vi "AlliGator Decay Fit Parameter Map Panel.vi"() -> ()   [LabVIEW 2021, in "AlliGator Decay Fit Parameter Map.lvlib"]
uses:
  AlliGator Decay Fit Parameter Map.lvlib
  Fits/IRF(X)PSED/Decay Fit Parameters & Derived Quantities List v2.ctl
  AlliGator Decay Fit Parameter Map Control Refnums.ctl
  Globals, Variables, Constants/AlliGator Refnums List.ctl
  Utilities/Read-Write.ctl
  Settings/AlliGator Settings List.ctl
  Action Engine/AlliGator Q Element.ctl
  Action Engine/AlliGator Q Event.ctl
  Globals, Variables, Constants/AlliGator Variables List.ctl
  Palette/Image Palette Information.ctl
  Image/Image Display Palette Type.ctl
  Image/Image Display Event.ctl
  Image/Image Control Refnum.ctl
  <vilib>/Utility/miscctls.llb/LVPoint32TypeDef.ctl
  AlliGator Decay Parameter Map Update Event Data.ctl
  GUI/AlliGator Image Mouse Up Event Data.ctl
  Image/Image ROI Descriptor.ctl
  Image/Image Contour Definition.ctl
  Image/Image Contour ID.ctl
  Image/Image ROI Type.ctl
  Variant/Variant to Data/Variant to Boolean.vi
  Variant/Variant to Data/Variant to [String].vi
  Settings/AlliGator Settings+.lvlib
  Variant/Variant to Data/Variant to Data.lvlib
  Notebook/Notebook.lvlib
  Action Engine/AlliGator Action Engine.lvlib
  GUI/GUI.lvlib
  GUI/AlliGator GUI.lvlib
  Error/Error.lvlib
  Image/Image.lvlib
  Palette/Palette.lvlib
  Globals, Variables, Constants/AlliGator Globals, Variables & Constants.lvlib
  Python Plugins API/AlliGator Python Plugins.lvlib
  Phasor Plot/AlliGator Phasor Plot.lvlib
  Fits/Fits.lvlib
  Utilities/Utilities.lvlib
panel:
  in  "Decay Fit Parameter":T1
  in  "Pin Button":bool=TRUE
  in  "Overlay Decay Fit Parameter Map":bool
  in  "Decay Fit Parameter ROI Color":u32(colorbox)=6618880 caption="Phasor Plot ROI Color"
  in  "Refresh Decay Fit Parameter Map":bool caption="Refresh Phsor Plot"
  out "Decay Fit Parameter Map Display":T2(plugin-control)
  out "Decay Parameter Map Value":dbl caption="Map Value" format="%#_5e"
  out "Decay Parameter Map Y":i32 caption="Y"
  out "Decay Parameter Map X":i32 caption="X"
  out "Decay Fit Min Parameter":dbl caption="Min Parameter" format="%#_5e"
  out "Decay Fit Max Parameter":dbl=1.0 caption="Max Parameter" format="%#_5e"
  in  "Decay Fit Parameter Map Color Scale":dbl(ramp)
  in  "Decay Fit Parameter Map Display Range":cluster{dbl, dbl}(slide)={0.0, 1.0} scale=0.7838060855865479..1.044173002243042 scale format="%04_3g"
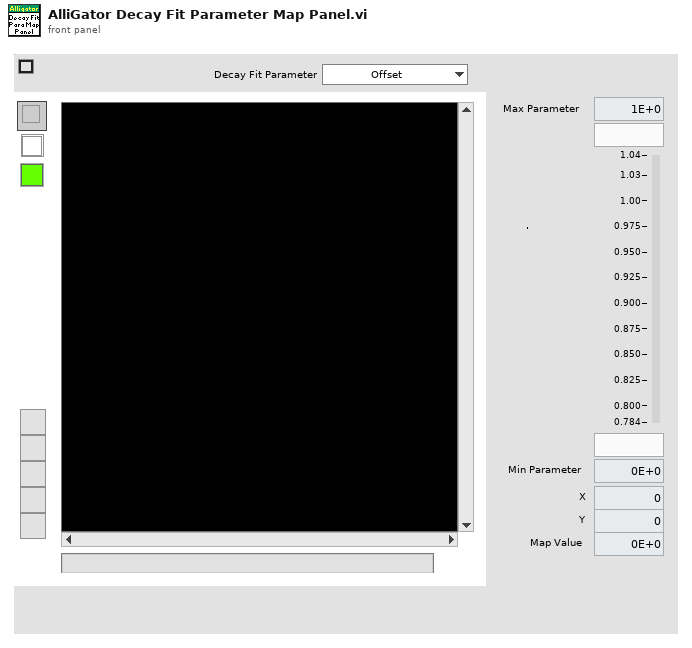
[diagram p1: front panel]
types:
  T1 = typedef "Fits.lvlib/Decay Fit Parameters & Derived Quantities List v2.ctl" = enum16{"Offset", "Baseline", "A_1", "tau_1", "A_2", "tau_2", "<tau>_a", "f1_a", "f2_a", "<tau>_i", "f1_i", "f2_i", "-", "R^2", "Chi^2"}
  T2 = typedef "IMAQ Image.ctl" = refnum<image>
  T3 = typedef "Utilities.lvlib/Read-Write.ctl" = enum16{"Read", "Write"}
  T4 = typedef "AlliGator GUI.lvlib/AlliGator Refnums List.ctl" = enum16{"---------- AlliGator Control Refnums ----------", "AlliGator Tab Control Refnum", "Dataset Ctrl Refnums", "Image Histogram Ctrl Refnums", "Intensity Time Trace Ctrl Refnums", "Decay Graph Ctrl Refnums", "Decay Statistics Graph Ctrl Refnums", "Phasor Graph Ctrl Refnums", "Phasor Ratio Graph Ctrl Refnums", "Phasor Plot Ctrl Refnums", "Lifetime & Other Parameters Ctrl Refnums", "Decay Fit Parameter Map Ctrl Refnums", "Parameter Map Ctrl Refnums", "Other AlliGator Ctrl Refnums", "---------- AlliGator Menu Refnums ----------", "AlliGator Menu", "---------- IO Device ID ----------", "Mouse ID", "Keyboard ID"}
  T5 = typedef "AlliGator Decay Fit Parameter Map.lvlib/AlliGator Decay Fit Parameter Map Control Refnums.ctl" = cluster{"Decay Fit Parameter Map Color Scale":refnum<vi>, "Decay Fit Parameter":refnum<vi>, "Max Parameter":refnum<vi>, "Min Parameter":refnum<vi>, "Decay Fit Parameter Map Display":refnum<vi>, "Decay Fit Parameter Map Display Range":refnum<vi>, "Decay Parameter Map X":refnum<vi>, "Decay Parameter Map Y":refnum<vi>, "Decay Parameter Map Value":refnum<vi>}
  T6 = cluster{"Event Registration Refnum":refnum<event-registration>, "Decay Fit Parameter Map Display Range Event":refnum<event-registration>, "Decay Fit Parameter Map Display Event":refnum<event-registration>}
  T7 = typedef "AlliGator Settings+.lvlib/AlliGator Settings List.ctl" = enum16{"GUI:Visible Settings Tab", "GUI:Last Run Version", "Source Image:Use Image Histogram for Contrast", "Source Image:Low Count Pixels Rejection Options", "Source Image:High Count Pixels Rejection Options", "Source Image:Use Image Brightness", "Source Image:Blend Overlay with Image Background", "Source Image:Use Fixed ROI Diameter", "Source Image:ROI Diameter", "Source Image:ROI Center Color", "Source Image:Peak Threshold", "Source Image:Intensity Threshold", "Source Image:Image Binning Options", "Source Image:Image Smoothing Options", "Source Image:Image Histogram Active", "Source Image:Invert Binary Mask", "Source Image:Hot Pixel Removal", "Source Image:Overlay Analyzed ROI Center", "Source Image:Auto-Adjust Contrast", "Source Image:Histogram Lower Percentile", "Source Image:Histogram Upper Percentile", "Source Image:Lock ROI with Maps", "Source Image:Save Source Image", "Source Image:Scale Bar Options", "Source Image:Image Resolution (Pixel Size)", "Source Image:Flatfield Correction", "Source Image:Show Dead Left Columns Correction", "Source Image:Dead Left Columns Correction", "Source Image:Image Pre-Processing Operations Order", "Source Image:Overlay ROI Median", "Source Image:Median Overlay Color", "Data Information:Gate Width", "Data Information:Nanotime Gate Separation", "Data Information:Macrotime Gate Separation", "Data Information:Gate Step", "Data Information:# Gates", "Data Information:Gate Image Exposure", "Data Information:Gate Image Integration", "Data Information:Gates to Skip", "Data Information:Gates to Keep", "Data Information:Define Gates to", "Data Information:Channel Name", "Data Information:Available Channel Names", "Data Information:Channel Arithmetic", "Data Information:Background File Subtraction", "Data Information:Background File", "Data Information:Background Scaling Factor", "Data Information:Background Pile-up Correction", "Data Information:Background Pixel Well Capacity", "Data Information:Laser Period", "Data Information:SYNC Period", "Data Information:Pile-up Correction", "Data Information:Pixel Well Capacity", "Data Information:Dataset Scaling Factor", "Fluorescence Decay_Decay Pre-Processing:Reverse Gates", "Fluorescence Decay_Decay Pre-Processing:Verbose Decay Pre-Processing", "Fluorescence Decay_Decay Pre-Processing:Use Decay Pre-Processing", "Fluorescence Decay_Decay Pre-Processing:Background Subtraction", "Fluorescence Decay_Decay Pre-Processing:Background Definition Range", "Fluorescence Decay_Decay Pre-Processing:Baseline Subtraction Method", "Fluorescence Decay_Decay Pre-Processing:Decay Pre-Processing Operations Order", "Fluorescence Decay_Decay Pre-Processing:Smoothing Parameter", "Fluorescence Decay_Decay Pre-Processing:Shift Decay", "Fluorescence Decay_Decay Pre-Processing:Decay Shift Parameters", "Fluorescence Decay_Decay Pre-Processing:Fold Decay", "Fluorescence Decay_Decay Pre-Processing:# Folds", "Fluorescence Decay_Decay Pre-Processing:1-Normalize Decay", "Fluorescence Decay_Decay Pre-Processing:[0-1]-Normalize Decay", "Fluorescence Decay_Decay Pre-Processing:Smoothen Decay", "Fluorescence Decay_Decay Pre-Processing:Extrapolate Decay", "Fluorescence Decay_Decay Pre-Processing:Use Periodicity", "Fluorescence Decay_Decay Pre-Processing:Use Cursors", "Fluorescence Decay_Decay Pre-Processing:Tail Fraction", "Fluorescence Decay_Decay Pre-Processing:Head Fraction", "Fluorescence Decay_Decay Pre-Processing:Additional Points", "Fluorescence Decay_Decay Pre-Processing:Straighten Decay", "Fluorescence Decay_Decay Pre-Processing:Constant Background", "Fluorescence Decay_Decay Pre-Processing:Pixel-Normalize Decay", "Fluorescence Decay_Advanced Analysis:Extract IRF instead of Decay", "Fluorescence Decay_Advanced Analysis:IRF Extraction Options", "Fluorescence Decay_Advanced Analysis:IRF Optimization Options", "Fluorescence Decay_Advanced Analysis:Square Pulse Options", "Fluorescence Decay_Advanced Analysis:IRF Order", "Fluorescence Decay_Advanced Analysis:IRF Time Constants", "Fluorescence Decay_Advanced Analysis:Wavelet Analysis Options", "Fluorescence Decay_Advanced Analysis:Average Lifetime Options", "Fluorescence Decay_Fit Options:Fit Options", "Fluorescence Decay_Fit Options:Use Legacy Fitting Approach", "Fluorescence Decay_Fit Options:Use Data Information Laser Period", "Fluorescence Decay_Fit Parameters:Displayed Fit Parameters", "Fluorescence Decay_Fit Parameters:Fit Parameter Constraints", "Fluorescence Decay_Fit Parameters:Export Tabulated Results", "Fluorescence Decay_Fit Parameters:MLE Baseline Offset Type", "Fluorescence Decay_Fit Parameters:MLE Baseline Offset", "Fluorescence Decay_Fit Parameters:Guess Parameter Names", "Fluorescence Decay_Fit Parameters:Guess Parameter Values", "Fluorescence Decay_Fit Parameters:Guess Parameters Options", "Fluorescence Decay_Fit Parameters:Optimal Offset Selection Criterion", "Fluorescence Decay_Styles:Show Last Decay Only", "Fluorescence Decay_Styles:Decay Graph Color Array", "Fluorescence Decay:Decay Graph Active", "Fluorescence Decay Statistics:Min Peak Value", "Fluorescence Decay Statistics:Reject Low Decay Peak Pixels", "Fluorescence Decay Statistics:Reject High Decay Peak Pixels", "Fluorescence Decay Statistics:Max Peak Value", "Time Traces:Use File Timestamp", "Time Traces:Time Step", "Time Traces:Use Intensity Correction File", "Time Traces:Intensity Correction File", "Phasor Plot:Phasor Plot Smoothing Options", "Phasor Plot:Phasor Plot Size", "Phasor Plot:Phasor Plot Graphics Options", "Phasor Plot:Cumulative Phasor Plot", "Phasor Plot:Use Phasor Brightness", "Phasor Plot:Blend Overlay with Phasor Background", "Phasor Plot:Save Phasor Plot", "Phasor Plot:Show References", "Phasor Plot:Phasor Ratio Decay Range", "Phasor Plot:Exponential Fading", "Phasor Plot:Phasor Ratio Reference Colors", "Phasor Plot:Reference Radius", "Phasor Plot:Show Color Map Vertices", "Phasor Plot:Phasor Plot Active", "Phasor Plot:Phasor Ratio Color Map Type", "Phasor Plot:Phasor Ratio Color Map", "Phasor Plot:Phasor Ratio Display Range", "Phasor Plot:Selected Image ROI(s)", "Phasor Plot:All Image ROIs", "Phasor Plot:Selected Phasor Plot ROI(s)", "Phasor Plot:All Phasor Plot ROIs", "Phasor Plot:Phasor Ratio Color-Coded Quantity", "Phasor Plot:Store Phasor Harmonics", "Phasor Plot:Draw Reference Segment", "Phasor Plot:User-Defined Quantity", "Phasor Plot:Color Scale High Color", "Phasor Plot:Color Scale Low Color", "Phasor Plot:Intensity-weighted Phasor Plot", "Phasor Graph:Phasor Frequency", "Phasor Graph:Phasor Ratio Type", "Phasor Graph:Pixel-level Phasor Computation", "Phasor Graph:Save Phasor Graph", "Phasor Graph:Phasor Graph Active", "Phasor Graph:Phasor SDV Options", "Phasor Graph:Intensity-weighted Phasor Graph", "Phasor Graph:Define Shortest Lifetime as", "Phasor Calibration:Use Backup Calibration if needed", "Phasor Calibration:Backup Calibration Type", "Phasor Calibration:Calibration Type", "Phasor Calibration:Calibration Lifetime", "Phasor Calibration:Calibration Map Algorithm", "Single-Exponential Phasor Locus (SEPL):Gate Parameters", "Single-Exponential Phasor Locus (SEPL):User-defined Gate", "Single-Exponential Phasor Locus (SEPL):User-defined IRF", "Single-Exponential Phasor Locus (SEPL):Phasor Parameters", "Single-Exponential Phasor Locus (SEPL):Decay & IRF Parameters", "Single-Exponential Phasor Locus (SEPL):Display Parameters", "Lifetime Analysis:Decay Analysis Parameters", "Lifetime Analysis:Lifetime Map Active", "Plugins:Python Settings", "Miscellaneous:Verbose Mode", "Miscellaneous:Beep after Script", "Miscellaneous:Saved Image File Format", "Miscellaneous:Exported Gate Image Settings", "Miscellaneous:Include Loading in Timing", "Miscellaneous:Verbose Settings Mode", "Miscellaneous:Histogram Options", "Miscellaneous:Beep on Error", "Miscellaneous:# Logical Processors Used", "Miscellaneous:ROI Description Max Characters", "Miscellaneous:Verbose Error Mode", "Miscellaneous:Transparent Mask Color"}
  T8 = typedef "AlliGator Action Engine.lvlib/AlliGator Q Element.ctl" = cluster{"AlliGator Q Event":T9, "Data":variant}
  T9 = typedef "AlliGator Action Engine.lvlib/AlliGator Q Event.ctl" = enum16{"---- Files ----", "Files:Set Batch Export Files To Save", "Files:Set Dataset Loading & Pre-processing Options", "Files:Check #Frames in Dataset", "Files:Increment Frame Index", "Files:Open Mask Image", "Files:Open White Light Image", "Files:Open Single Dataset", "Files:New Folder of Folders Selected", "Files:Load File (all Types)_Scriptable", "Files:Move Flattened Series to Folders Series", "Files:Select Folder", "Files:Load FLI Dataset", "Files:Load Swiss SPAD 1 Dataset", "Files:Load Swiss SPAD 2 Dataset", "Files:Load .sdt FLI Dataset", "Files:Load .ptu FLI Dataset", "Files:Load .bin FLI Dataset", "Files:Load Single Gate Image Folder", "Files:Load I/m/phi Dataset (deprecated)", "Files:Load Single Image", "Files:Subtract Background File", "Files:Export FLI Dataset", "Files:Load HDF5 FLI Dataset", "Files:Set Destination File Path", "Files:Save Mask Image", "Files:Batch Conversion", "Files:New Folder Selected", "Files:Close FLI Dataset", "Files:Close FLI Dataset Series", "Files:Close White Light Image", "Files:Close Mask Image", "---- FLI Dataset ----", "FLI Dataset:Channel Arithmetic", "FLI Dataset:Export Average Lifetime Map as ASCII", "FLI Dataset:Export User-Defined Quantity Map as ASCII", "FLI Dataset:Python Function FLI Dataset Event", "FLI Dataset:ROI Analysis", "FLI Dataset:Tilted Logistic Square Gated IRF Characteristics Map", "FLI Dataset:Logistic Square Gated IRF Characteristics Map", "FLI Dataset:Square Gated IRF Characteristics Map", "FLI Dataset:Multi-ROI Single-Pixel Phasor Analysis", "FLI Dataset:Multi-ROI Single-Pixel NLSF Analysis", "FLI Dataset:All ROIs IRF Extraction", "FLI Dataset:All ROIs Decay Fit Non-Interactive (Fast + Individual IRF)", "FLI Dataset:All ROIs Phasor Analysis", "FLI Dataset:All ROIs Decay Fit", "FLI Dataset:Fluorescence Decay Statistics", "FLI Dataset:Update Decay Statistics Graph", "FLI Dataset:Get Decay from ROI", "FLI Dataset:All ROIs Average Lifetimes", "FLI Dataset:Save/Load Local IRFs", "FLI Dataset:Clear Local IRFs", "FLI Dataset:Phasor Calibration Maps (# Gates Series) Script", "FLI Dataset:Calibrated Phasor Map Series", "---- FLI Dataset Series ----", "FLI Dataset Series:Sum All Datasets in Series", "FLI Dataset Series:Add Dataset to Accumulated Dataset", "FLI Dataset Series:Display Accumulated Dataset", "FLI Dataset Series:Clear Dataset Series Sum", "FLI Dataset Series:Time-Series Analysis (NLSF)", "FLI Dataset Series:Time-Series Analysis (Phasor)", "---- Image ----", "Image:Update Image Profile Plots", "Image:Image Histogram Cursor Move", "Image:Image Histogram", "Image:Image Contrast", "Image:Set Image Histogram Cursor Move Flag", "Image:Clear Image Overlay", "Image:Use ROI as Search Area", "Image:Set ROI Diameter", "Image:Save Image Data as TIFF", "Image:Save Displayed Image with Overlay", "Image:Save Image Overlay Only", "Image:Save Image as Hot Pixel Mask", "Image:Change Source Image Color Palette", "Image:Copy Image to Clipboard", "Image:Source Image ROI Selection", "Image:Delete All ROIs", "Image:Delete All Unselected ROIs", "Image:Delete ROI", "Image:Merge All ROIs", "Image:Store ROI", "Image:Source Image ROI Storage", "Image:Export ROI Description to Notebook", "Image:Save ROI", "Image:Load ROI", "Image:Paste ROI Definition", "Image:Clear ROI", "Image:Identify ROIs in Mask Image", "Image:Create Complementary ROI", "Image:Create Contour ROI", "Image:Create ROI(s) from Pixels with Peak above Min_Scriptable", "Image:Create ROI(s) from Pixels with Intensity above Min_Scriptable", "Image:Compute ROI Statistics", "Image:Delete ROI(s) based on ROI Characteristics", "Image:Create ROI Grid", "Image:ROI to Individual Pixel ROIs", "Image:Python Function Source Image Event", "Image:Show Phasor Calibration Map ROI Centers", "Image:Convert ROI to Mask Image", "Image:Mouse Move", "Image:Mouse Up", "Image:Set Source Image Mouse Move Flag", "Image:Add Scale Bar Overlay", "Image:Delete Existing ROIs Option", "Image:Overlay ROI Median", "Image:Check Current ROI", "Image:Update True Pixel Value", "Image:Use ROI", "---- Decay ----", "Decay:Clear IRF/Reference Plot", "Decay:Add Decay to Graph", "Decay:Smoothen Plot", "Decay:Smoothen Plot Tail", "Decay:Average Selected Plots", "Decay:Extract IRF", "Decay:Optimal IRF Extraction", "Decay:Threshold IRF", "Decay:Fit to Model IRF", "Decay:Fit IRF to Square Gate", "Decay:Fit IRF to Logistic Square Gate", "Decay:Fit IRF to Tilted Logistic Square Gate", "Decay:Create Bounding Cursors Set", "Decay:Export Bounding Cursors Definition to Notebook", "Decay:Denoise Plot", "Decay:Compute Cumulative Function", "Decay:Use as Reference Decay", "Decay:Show Reference Decay/IRF", "Decay:Extrapolate Decay", "Decay:Create Head & Tail Bounding Cursors", "Decay:Store Cursor-defined Head & Tail Fractions", "Decay:Rebin Plot", "Decay:1-Normalize Decay", "Decay:[0-1]-Normalize Plot", "Decay:Straighten Decay", "Decay:Shift Decay", "Decay:Fold Decay", "Decay:Fit Decay", "Decay:Global Fit of Selected Decays", "Decay:Post Global Fit Script", "Decay:Add Global Fit Parameters to Graph", "Decay:Add Decay Parameter(s) to Plot (Graph)", "Decay:Export Decay to Phasor Graph", "Decay:Compute Average Lifetime", "Decay:Plot Convolution", "Decay:Graph Tip Strip Update", "---- Decay Statistics ----", "Decay Statistics:Tip Strip Update", "---- Intensity Time Trace ----", "Intensity Time Trace:Use File Timestamp", "Intensity Time Trace:Load Intensity Corrections File", "Intensity Time Trace:Clear Intensity Corrections File", "Intensity Time Trace:Tip Strip Update", "---- Phasor Plot ----", "Phasor Plot:Build Phasor Plot", "Phasor Plot:Change Phasor Plot Color Palette", "Phasor Plot:Adjust Phasor Plot Display Range", "Phasor Plot:Highlight Image ROI in Phasor Plot", "Phasor Plot:Save Phasor Plot Image with Overlay", "Phasor Plot:Export Complex Phasor Map", "Phasor Plot:Export Phasor Ratio Map", "Phasor Plot:Export Average Lifetime Map", "Phasor Plot:Compute Phase Lifetime Histogram", "Phasor Plot:Compute Phasor Ratio Histogram", "Phasor Plot:Compute Phase Lifetime vs Intensity Scatter Plot", "Phasor Plot:Weber 2-Component Decomposition", "Phasor Plot:Update Phasor Color Map Vertices", "Phasor Plot:Clear Phasor Overlay", "Phasor Plot:Use Segment Extremities as References", "Phasor Plot:Use UC/Segment Intersections as References", "Phasor Plot:Use UC/Principal Axis Intersections as References", "Phasor Plot:Use UC/Linear Fit Intersections as References", "Phasor Plot:Update Phasor Plot Reference", "Phasor Plot:Show Local Phasor Info in Phasor Plot", "Phasor Plot:Update Phasor Plot State", "Phasor Plot:Phasor Plot ROI Storage", "Phasor Plot:Phasor Plot ROI Selection", "Phasor Plot:Python Function Phasor Plot Event", "Phasor Plot:Overlay Phasor ROI, Ratio or Map in Source Image", "Phasor Plot:Compute Decay of Selected Phasors", "Phasor Plot:Phasor at Image Pixel", "Phasor Plot:Mouse Move", "Phasor Plot:Mouse Up", "Phasor Plot:Display Range Mouse Move", "Phasor Plot:Set Mouse Move Flag", "Phasor Plot:Update True Phasor Plot Value", "---- Phasor Graph ----", "Phasor Graph:Get Phasor Value", "Phasor Graph:Create New Phasor Plot Dialog", "Phasor Graph:Update Last Phasor Value", "Phasor Graph:Update Phasor (m, phi)", "Phasor Graph:Remove Single Phasor from Plot", "Phasor Graph:Add Single Phasor to Plot", "Phasor Graph:Remove Phasor Plot", "Phasor Graph:Remove Selected Phasor Plots", "Phasor Graph:Clear Phasor Data", "Phasor Graph:Clear Phasor Graph", "Phasor Graph:Cursor Move", "Phasor Graph:Draw Cursor Connecting Line", "Phasor Graph:Clear Cursor Connecting Line", "Phasor Graph:Find UC Intersection", "Phasor Graph:Use UC/Cursor-Defined Line Intersections", "Phasor Graph:Use Selected Plots Fitted Line/UC Intersections", "Phasor Graph:Use Selected Plots Principal Axis/UC Intersections", "Phasor Graph:Show Single Phasor", "Phasor Graph:Save Single Phasor Plot", "Phasor Graph:Save All Phasor Plots", "Phasor Graph:Load Phasor Plot(s)", "Phasor Graph:Phasor Multiplication", "Phasor Graph:Compute Average Phasor", "Phasor Graph:Compute Multiple Average Phasors (Selected Plots)", "Phasor Graph:Export Single Phasor Plot Phase Lifetimes", "Phasor Graph:Parameter 2 vs Parameter 1 Scatter Plot", "Phasor Graph:Use Cursor n Location", "Phasor Graph:Set Reference n to Current Phase Lifetime Value", "Phasor Graph:Set Reference n to Lifetime Value", "Phasor Graph:Set Cursor n Location", "Phasor Graph:Save Phasor Graph Image", "Phasor Graph:Update SEPL Plot", "Phasor Graph:Export Single Phasor Plot Data", "Phasor Graph:Export Selected Phasor Plots Data", "Phasor Graph:Python Function Phasor Graph Event", "Phasor Graph:Tip Strip Update", "---- Calibration ----", "Calibration:Set Calibration Type", "Calibration:Load/Save Phasor Calibration", "Calibration:Load/Save Phasor Calibration Series", "Calibration:Load/Save Phasor Calibration Map", "Calibration:Use as Calibration", "Calibration:Compute Optimal Calibration from Phasor References", "Calibration:Clear Phasor Calibration", "Calibration:Single Phasor Calibration Information", "Calibration:Use as Calibration Series", "Calibration:Use as Calibration Map", "Calibration:Clear Calibration Series", "Calibration:Phasor Calibration Series Information", "Calibration:Clear Calibration Map", "Calibration:Phasor Calibration Map Information", "Calibration:Apply Phasor Calibration", "Calibration:Update Single Plot Calibration", "Calibration:Update Multiple Plots Calibration", "Calibration:Clear Single Plot Calibration", "Calibration:Clear All Plots Calibrations", "Calibration:Clear Plot(s) Calibration(s)?", "---- Phasor Ratio ----", "Phasor Ratio:Clear Reference n", "Phasor Ratio:Toggle Selected Plot(s)  Lock to Reference 1", "Phasor Ratio:Use as Reference n", "Phasor Ratio:Send Reference n to Notebook", "Phasor Ratio:Toggle Selected Plot(s)  Lock to Reference 2", "Phasor Ratio:Compute Phasor Ratio at Mouse Location", "Phasor Ratio:Compute Phasor Plot's Average Phasor Ratio", "Phasor Ratio:Compute Time-Series Phasor Ratios", "Phasor Ratio:Fit Line to Phasor Ratio Plot", "Phasor Ratio:Save References", "Phasor Ratio:Load References", "Phasor Ratio:Update Phasor Reference 1", "Phasor Ratio:Update Phasor Reference 2", "Phasor Ratio:Move Cursor n to Reference n", "Phasor Ratio:Use as Phasor Reference 1 Lifetime", "Phasor Ratio:Use as Phasor Reference 2 Lifetime", "Phasor Ratio:Export Phasor Ratio Map as ASCII", "Phasor Ratio:Tip Strip Update", "---- Lifetime & Other Parameters Graph ----", "Lifetime:Compute Sliced Mean, SDV and CV Plots", "Lifetime:Plot Decay Shifts", "Lifetime:Plot Histogram", "---- Decay Fit Parameter Map ----", "Decay Fit Parameter Map:Export ROI NLSF Data as ASCII", "Decay Fit Parameter Map:Set Decay Fit Parameter Map Selection", "Decay Fit Parameter Map:Build Decay Fit Parameter Map", "Decay Fit Parameter Map:Change Decay Fit Parameter Map Color Palette", "Decay Fit Parameter Map:Export Decay Fit Parameter Map Data as ASCII", "Decay Fit Parameter Map:Export All Decay Fit Parameter Maps Data as ASCII", "Decay Fit Parameter Map:Selected Parameter Scatterplot", "Decay Fit Parameter Map:Parameter 2 vs Parameter 1 Scatterplot", "Decay Fit Parameter Map:Save Decay Fit Parameter Map Image", "Decay Fit Parameter Map:Save-Load IRFs & Fit Data", "Decay Fit Parameter Map:Update Local Decay Plots", "Decay Fit Parameter Map:Python Function Decay Fit Parameters Map Event", "Decay Fit Parameter Map:Overlay Decay Fit Parameter Map in Source Image", "Decay Fit Parameter Map:Selected Parameter vs Intensity Scatterplot", "Decay Fit Parameter Map:Mouse Up", "Decay Fit Parameter Map:Mouse Move", "Decay Fit Parameter Map:Display Range Mouse Move", "Decay Fit Parameter Map:Change Map Resolution", "Decay Fit Parameter Map:Variance Significance Maps", "Decay Fit Parameter Map:Fit Result Constraints Window", "Decay Fit Parameter Map:Use ROI", "---- Parameter Map ----", "Parameter Map:Export ROI Parameters Data as ASCII", "Parameter Map:Add Parameter Map Set", "Parameter Map:Delete Parameter Map Set", "Parameter Map:Update Parameter List", "Parameter Map:Build Parameter Map", "Parameter Map:Change Parameter Map Color Palette", "Parameter Map:Export Parameter Map Data as ASCII", "Parameter Map:Export All Parameter Maps Data as ASCII", "Parameter Map:Selected Parameter Scatterplot", "Parameter Map:Parameter 2 vs Parameter 1 Scatterplot", "Parameter Map:Selected Parameter vs Intensity Scatterplot", "Parameter Map:Save Parameter Map Image", "Parameter Map:Save-Load IRFs & Parameter Maps (TODO)", "Parameter Map:Set Parameter Map Selection", "Parameter Map:Python Function Parameter Map Event", "Parameter Map:Overlay Parameter Map in Source Image", "Parameter Map:Update Local Decay Plots", "Parameter Map:Mouse Up", "Parameter Map:Mouse Move", "Parameter Map:Display Range Mouse Move", "Parameter Map:Use ROI", "---- Generic Graph ----", "Generic Graph:Generic XY Graph Event", "Generic Graph:Python Function XY Graph Event", "Generic Graph:New Plot", "Generic Graph:Save Plot", "Generic Graph:XY Plot Histogram", "Generic Graph:Set XY Graph Plot Name", "Generic Graph:Set Last Cursor Style", "Generic Graph:Tip Strip Update", "---- GUI ----", "GUI:Start Script", "GUI:Type of Displayed Image Changed", "GUI:Gate Image Slide Changed", "GUI:Show Busy Icon", "GUI:Show Busy Icon & Abort Button", "GUI:Hide Busy Icon", "GUI:Hide Busy Icon & Abort Button", "GUI:Abort", "GUI:End Script", "GUI:Start Timing", "GUI:End Timing", "GUI:Set State Indicator", "GUI:Send Parameters JSON Strings to Clipboard", "GUI:Set Gate Step", "GUI:Idle", "GUI:Initialization", "GUI:Quit", "GUI:Increment Dataset Index", "GUI:Set Dataset Index to -1", "GUI:Time Series Slider Moved", "GUI:Time Series Slider Changed", "GUI:Toggle Playback or Loop", "GUI:Playback Script", "GUI:Set Phasor Frequency", "GUI:Open Window", "GUI:Start Test Script", "GUI:End Test Script", "GUI:Set Verbose Mode", "GUI:Set Verbose Settings Mode", "GUI:Initialize Python Session", "DEBUG"}
  T10 = typedef "Palette.lvlib/Image Palette Information.ctl" = cluster{"Palette Name [# Colors,int?,inv?]":string, "Palette Type":T11, "Palette Colors":u32[], "Interpolate?":bool}
  T11 = typedef "Image.lvlib/Image Display Palette Type.ctl" = u32
  T12 = typedef "AlliGator Globals, Variables & Constants.lvlib/AlliGator Variables List.ctl" = enum16{"---- GUI ----", "GUI:Initialization Status", "GUI:State Indicators Refnum", "GUI:Original AlliGator Menu Items", "GUI:Current Action Loop State", "GUI:Script in progress", "GUI:Playback", "GUI:Loop Playback", "GUI:Search ROI Used", "GUI:Search ROI", "Image Histogram Max Legend Size", "Decay Graph Max Legend Size", "Intensity Graph Max Legend Size", "Decay Statistics Graph Max Legend Size", "Phasor Graph Max Legend Size", "Phasor Ratio Graph Max Legend Size", "Lifetime Graph Max Legend Size", "---- Files ----", "Files:Export Dataset Frames as Individual Files", "Files:Show Batch Export Help Balloons", "Files:Frames in Dataset", "Files:ptu File Frame Start Indices", "Files:Current Frame in Dataset", "Files:Current Frame Timestamp", "Files:Dataset Loaded", "Files:Dataset Metadata", "Files:Dataset Channel", "Files:Dataset Data Description", "Files:Background Dataset Metadata", "Files:Background Dataset Channel", "Files:Background Dataset Data Description", "Files:Background File Subtraction", "Files:Background File Path", "Files:Background File Pile-up Correction", "Files:Background File Pixel Well Capacity", "Files:Background File Scaling Factor", "Files:Current Dataset Load Settings", "Files:Dataset Path", "Files:ICCD-specific Information", "Files:Macrotime Gate Separation", "------ Python Plugins ------", "Python Plugins:Information", "Python Plugins:Python Session", "Python Plugins:Valid Python Session?", "---- Source Image ----", "Source Image:ROIs", "Source Image:Current ROI", "Source Image:ROI Event Refnum", "X_Source Image:Display Range", "X_Source Image:Palette Information", "X_Source Image:Type of Displayed Image", "X_Time Gate Slider", "Source Image:Palette List", "Source Image:Scale", "Source Image:ROI Overlay Color", "Source Image:Overlay to Erase", "Source Image:Is Displayed Image Accumulated", "Source Image:White Light Image Modified", "Source Image:Mask Image Modified", "---- Image Profile Window ----", "Image Profile:Window Event Refnum", "Image Profile:IntensityType", "Image Profile:Intensity Average Type", "Image Profile:Intensity-weighted SDV", "Image Profile:Box Profile Type", "Image Profile:Window Open", "Image Profile:Plotted Fit Parameter", "------ Phasor Graph -------", "Phasor Graph:Show Line", "---- Phasor Plot ---", "Phasor Plot:Parameters Changed", "Phasor Plot:FLI Dataset Modified since last Calculation", "Phasor Harmonics Data", "Selected Phasor Harmonics", "Phasor Harmonic Manager Event Refnum", "Phasor Plot:ROIs", "Phasor Plot:Current ROI", "Phasor Plot:ROI Event Refnum", "Phasor Plot:Image Reference Points", "Phasor Plot:Computed", "Phasor Plot:Palette Information", "Phasor Plot:Palette List", "Phasor Plot:Phasor Ratio Palette Information", "Phasor Plot:Phasor Ratio Palette List", "Phasor Plot:Image Scale", "Phasor Plot:Image Overlay to Erase", "Phasor Plot:Image Elements to Update", "Phasor Plot:Current Calculation Parameters", "Phasor Plot:Current Calibration Options", "Phasor Plot:Reset Cumulated Phasor Plot", "Phasor Plot:Reference 1", "Phasor Plot:Lifetime Reference 1", "Phasor Plot:Reference 1 Frequency", "Phasor Plot:Reference 2", "Phasor Plot:Lifetime Reference 2", "Phasor Plot:Reference 2 Frequency", "---- Decay Analysis ----", "Number of Selected Decays to Fit", "LS Fit Results", "LAR Fit Results", "BS Fit Results", "Last Decay Max - Min", "Best Fit Parameters", "Best Fit Parameter Names", "Actual Size X", "Actual Size Y", "Binning X", "Binning Y", "Actual # Gates", "Dataset Number", "Gates to...", "Gates Skipped", "Gates to keep", "Gate Step", "Gate Separation", "Reversed Gates", "Pile-up Correction", "Pixel Well Capacity", "Background Subtracted", "Background Subtraction Method", "Background Definition Range", "Background File (deprecated)", "Number of Dataset Accumulated", "Array of Accumulated Dataset Paths", "Do Averaged Datasets", "Destination File Path", "Process Plot Target", "Use 1/D as Phasor Frequency", "---- Decay Fit Parameter Map -----", "Decay Fit Parameter Map:Palette Information", "Decay Fit Parameter Map:Palette List", "Decay Fit Parameter Map:X Resolution", "Decay Fit Parameter Map:Y Resolution", "Decay Fit Parameter Map:Use Decay Fit Result Constraints", "Decay Fit Parameter Map:Decay Fit Result Constraints", "Decay Fit Parameter Map:Decay Fit Result Constraints Applied", "---- Parameter Map ----", "Parameter Map:Palette Information", "Parameter Map:Palette List", "------- Local Decay Window ---------", "Local Decay Graph Window:Event Refnum", "Local Decay Graph Window:Use normalized IRF for convolution", "----- Miscellaneous ----", "Misc:Skippable Dialog Windows Status"}
  T13 = enum16{"0", "1", "2", "3", "4", "5", "6", "7", "8", "9", "A", "B", "C", "D", "E", "F", "G", "H", "I", "J", "K", "L", "M", "N", "O", "P", "Q", "R", "S", "T", "U", "V", "W", "X", "Y", "Z", "F1", "F2", "F3", "F4", "F5", "F6", "F7", "F8", "F9", "F10", "F11", "F12", "F13", "F14", "F15", "ADD", "BACK", "BACKSLASH", "CAPITAL", "COMMA", "DECIMAL", "DELETE", "DIVIDE", "DOWN", "END", "EQUALS", "ESCAPE", "GRAVE (`)", "HOME", "INSERT", "LBRACKET", "LCONTROL", "LEFT", "L ALT", "LSHIFT", "LWIN", "MINUS", "MULTIPLY", "NEXT", "NUMLOCK", "NUMPAD_0", "NUMPAD_1", "NUMPAD_2", "NUMPAD_3", "NUMPAD_4", "NUMPAD_5", "NUMPAD_6", "NUMPAD_7", "NUMPAD_8", "NUMPAD_9", "PAUSE", "PERIOD", "PRIOR (PG UP)", "RBRACKET", "RCONTROL", "RETURN", "RIGHT", "R ALT", "RSHIFT", "RWIN", "SCROLL", "SEMICOLON", "SLASH", "SPACE", "SUBTRACT", "TAB", "UP", "ENTER (num pad)", "' (quote)"}
  T14 = typedef "Image.lvlib/Image Display Event.ctl" = cluster{"Item Tag":string, "Image Control Refnum":T15, "Coords":T16, "Item Path":string}
  T15 = typedef "Image.lvlib/Image Control Refnum.ctl" = refnum<vi>
  T16 = typedef "LVPoint32TypeDef.ctl" = cluster{"Horizontal":i32, "Vertical":i32}
  T17 = typedef "AlliGator Decay Fit Parameter Map.lvlib/AlliGator Decay Parameter Map Update Event Data.ctl" = cluster{"Parameter":T1, "Parameter changed":bool}
  T18 = typedef "AlliGator GUI.lvlib/AlliGator Image Mouse Up Event Data.ctl" = cluster{"Current ROI Tool":u32, "ROI Descriptor":T19, "Shift":bool, "Alt":bool, "Image Display Refnum":T15}
  T19 = typedef "Image.lvlib/Image ROI Descriptor.ctl" = cluster{"Global Rectangle":i32[], "Contours":T20[]}
  T20 = typedef "Image.lvlib/Image Contour Definition.ctl" = cluster{"Contour Type":T21, "ROI Type":T22, "Points":i32[]}
  T21 = typedef "Image.lvlib/Image Contour ID.ctl" = enum32{"External", "Internal"}
  T22 = typedef "Image.lvlib/Image ROI Type.ctl" = enum16{"No Selection", "Point", "Line", "Rectangle", "Oval", "Polygon", "Freehand Region", "Annulus", "Unused2", "Unused3", "Broken Line", "Freehand Line", "Rotated Rectangle"}
  T23 = enum16{"0", "1", "2", "3", "4", "5", "6", "7", "8", "9", "A", "B", "C", "D", "E", "F", "G", "H", "I", "J", "K", "L", "M", "N", "O", "P", "Q", "R", "S", "T", "U", "V", "W", "X", "Y", "Z", "F1", "F2", "F3", "F4", "F5", "F6", "F7", "F8", "F9", "F10", "F11", "F12", "F13", "F14", "F15", "ADD", "BACK", "BACKSLASH", "CAPITAL", "COMMA", "DECIMAL", "DELETE", "DIVIDE", "DOWN", "END", "EQUALS", "ESCAPE", "GRAVE (`)", "HOME", "INSERT", "LBRACKET", "LCONTROL", "LEFT", "L ALT", "LSHIFT", "LWIN", "MINUS", "MULTIPLY", "NEXT", "NUMLOCK", "NUMPAD_0", "NUMPAD_1", "NUMPAD_2", "NUMPAD_3", "NUMPAD_4", "NUMPAD_5", "NUMPAD_6", "NUMPAD_7", "NUMPAD_8", "NUMPAD_9", "PAUSE", "PERIOD", "PRIOR (PG UP)", "RBRACKET", "RCONTROL", "RETURN", "RIGHT", "R ALT", "RSHIFT", "RWIN", "SCROLL", "SEMICOLON", "SLASH", "SPACE", "SUBTRACT", "TAB", "UP", "ENTER (num pad)", "' (quote)"}[]
  T24 = cluster{"button 1":bool, "button 2":bool, "button 3":bool, "button 4":bool}
  T25 = cluster{"Global Rectangle":i32[], "Contours":cluster{"Contour Type":u32, "ROI Type":u32, "Points":i32[]}[]}
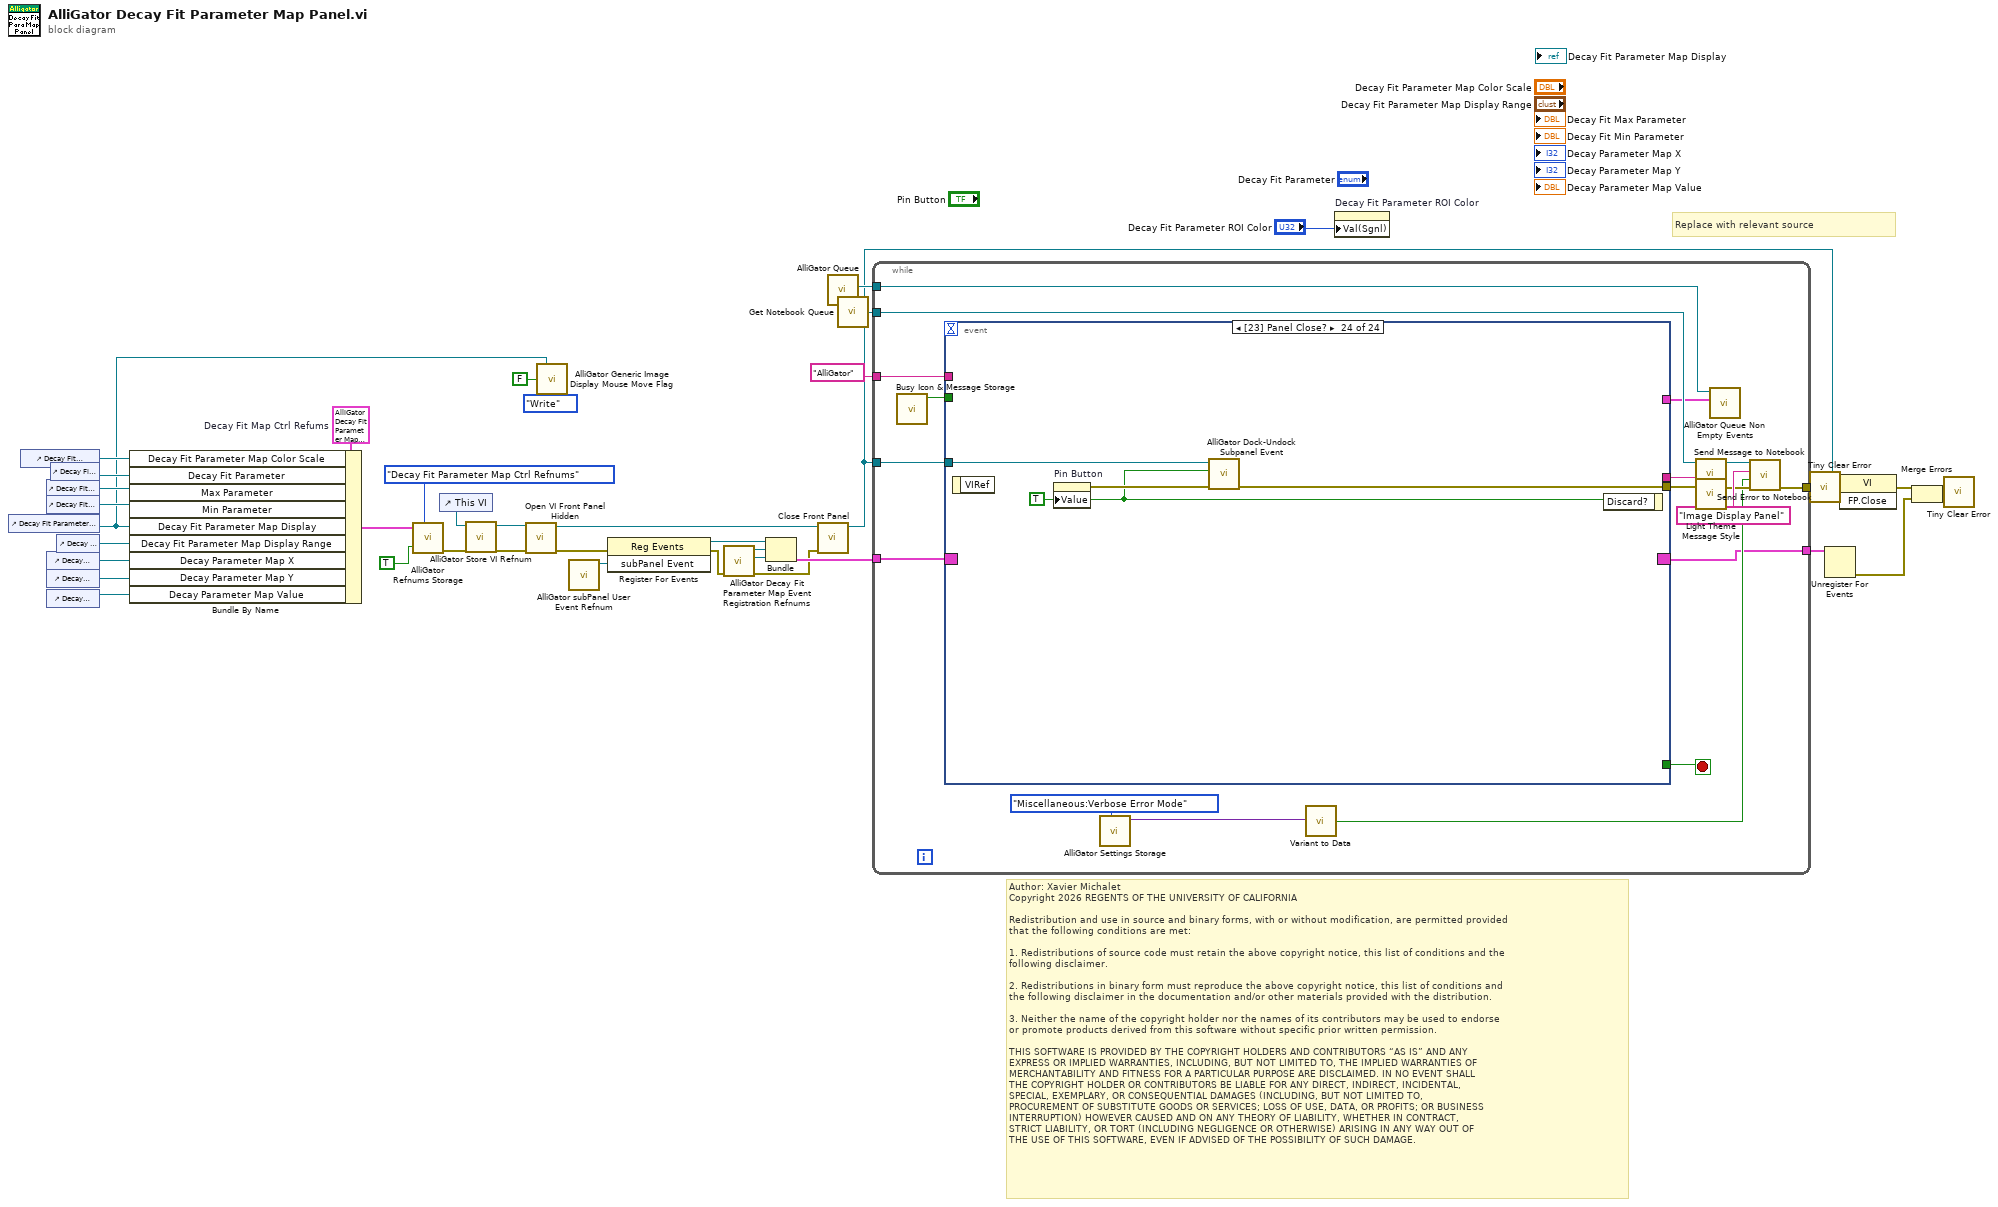
[diagram p0: block diagram]
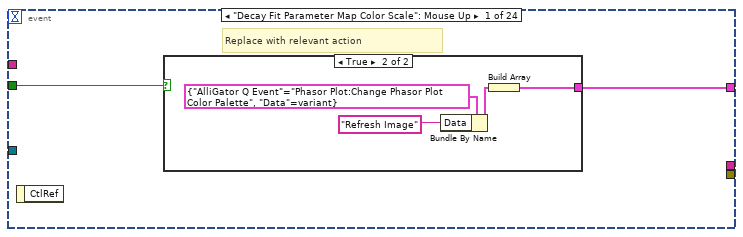
[diagram p2: hidden frame]
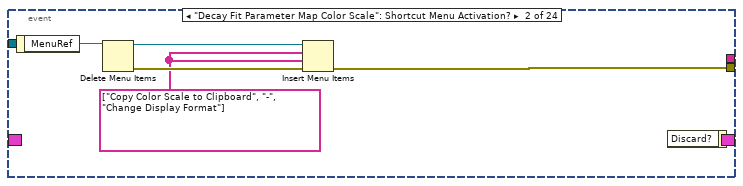
[diagram p4: hidden frame]
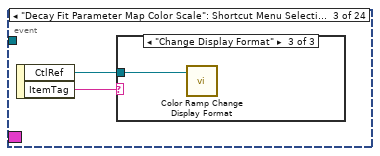
[diagram p5: hidden frame]
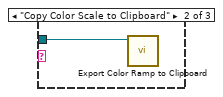
[diagram p7: hidden frame]
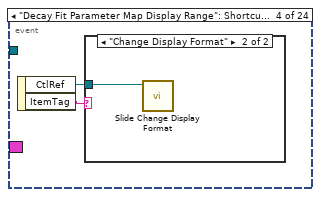
[diagram p8: hidden frame]
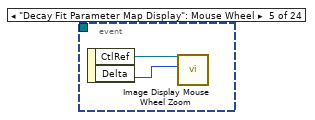
[diagram p10: hidden frame]
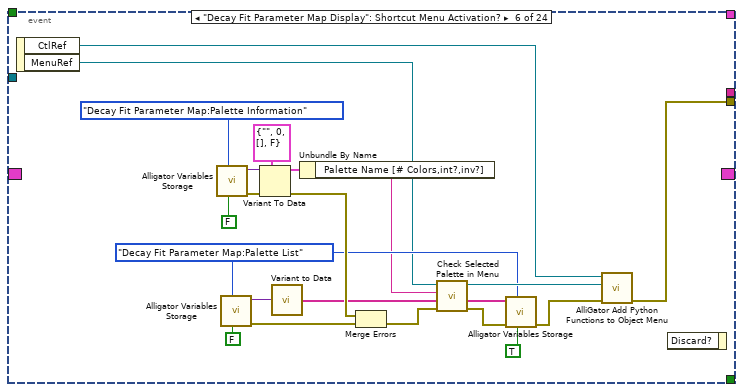
[diagram p11: hidden frame]
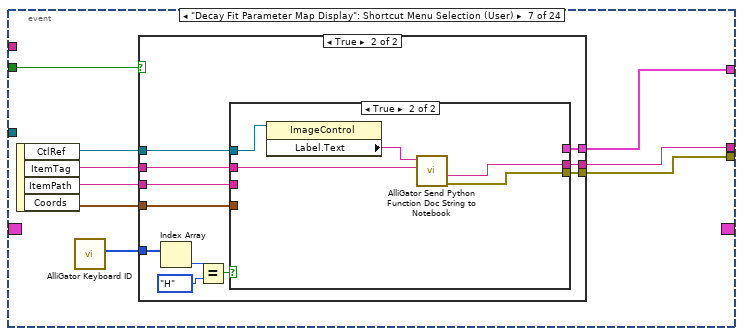
[diagram p12: hidden frame]
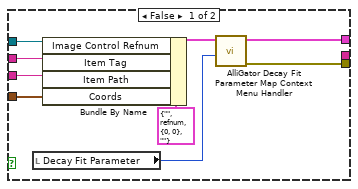
[diagram p14: hidden frame]
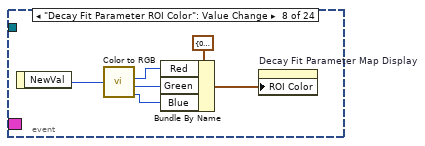
[diagram p15: hidden frame]
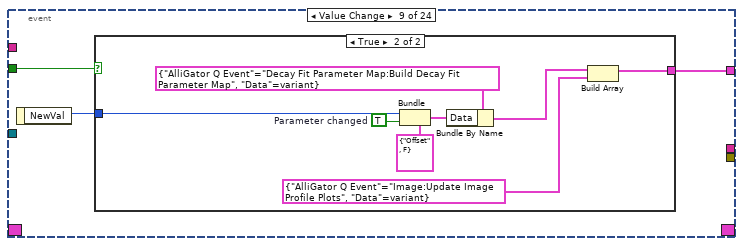
[diagram p16: hidden frame]
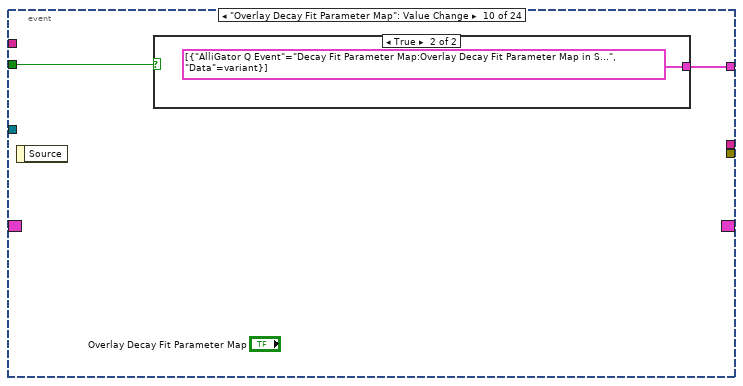
[diagram p18: hidden frame]
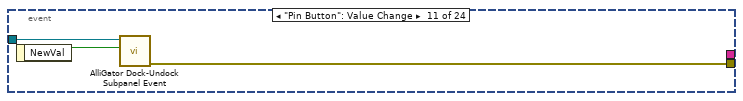
[diagram p20: hidden frame]
diagram:
  w23 = T5 {"Decay Fit Parameter Map Color Scale"=refnum, "Decay Fit Parameter"=refnum, "Max Parameter"=refnum, "Min Parameter"=refnum, "Decay Fit Parameter Map Display"=refnum, "Decay Fit Parameter Map Display Range"=refnum, "Decay Parameter Map X"=refnum, "Decay Parameter Map Y"=refnum, "Decay Parameter Map Value"=refnum}  # Decay Fit Map Ctrl Refums
  # "Replace with relevant source"
  # "Author: Xavier Michalet\nCopyright 2026 REGENTS OF THE UNIVERSITY OF CALIFORNIA\n\nRedistribution and use in source and binary forms, with or without modification, are permitted provided\nthat the following conditions are met:\n\n1. Redistributions of source code must retain the above copyright notice, this list of conditions and the\nfollowing disclaimer.\n\n2. Redistributions in binary form must reproduce the above copyright notice, this list of conditions and\nthe following disclaimer in the documentation and/or other materials provided with the distribution.\n\n3. Neither the name of the copyright holder nor the names of its contributors may be used to endorse \nor promote products derived from this software without specific prior written permission.\n\nTHIS SOFTWARE IS PROVIDED BY THE COPYRIGHT HOLDERS AND CONTRIBUTORS “AS IS” AND ANY \nEXPRESS OR IMPLIED WARRANTIES, INCLUDING, BUT NOT LIMITED TO, THE IMPLIED WARRANTIES OF\nMERCHANTABILITY AND FITNESS FOR A PARTICULAR PURPOSE ARE DISCLAIMED. IN NO EVENT SHALL\nTHE COPYRIGHT HOLDER OR CONTRIBUTORS BE LIABLE FOR ANY DIRECT, INDIRECT, INCIDENTAL, \nSPECIAL, EXEMPLARY, OR CONSEQUENTIAL DAMAGES (INCLUDING, BUT NOT LIMITED TO, \nPROCUREMENT OF SUBSTITUTE GOODS OR SERVICES; LOSS OF USE, DATA, OR PROFITS; OR BUSINESS\nINTERRUPTION) HOWEVER CAUSED AND ON ANY THEORY OF LIABILITY, WHETHER IN CONTRACT, \nSTRICT LIABILITY, OR TORT (INCLUDING NEGLIGENCE OR OTHERWISE) ARISING IN ANY WAY OUT OF\nTHE USE OF THIS SOFTWARE, EVEN IF ADVISED OF THE POSSIBILITY OF SUCH DAMAGE."
  n1 = control-ref of="Decay Fit Parameter Map Display"() -> (w5:refnum<vi>)
  n2 = control-ref of="Decay Fit Parameter Map Color Scale"() -> (w22:refnum<vi>)
  n3 = control-ref of="Decay Fit Max Parameter"() -> (w15:refnum<vi>)
  n4 = control-ref of="Decay Fit Min Parameter"() -> (w20:refnum<vi>)
  n5 = control-ref of="Decay Parameter Map X"() -> (w19:refnum<vi>)
  n6 = control-ref of="Decay Parameter Map Y"() -> (w18:refnum<vi>)
  n7 = control-ref of="Decay Parameter Map Value"() -> (w17:refnum<vi>)
  n8 = control-ref of="Decay Fit Parameter"() -> (w16:refnum<vi>)
  n9 = control-ref of="Decay Fit Parameter Map Display Range"() -> (w21:refnum<vi>)
  n10 = Bundle By Name(cluster=w23, "Decay Fit Parameter Map Color Scale"=w22, "Decay Fit Parameter"=w16, "Max Parameter"=w15, "Min Parameter"=w20, "Decay Fit Parameter Map Display"=w5, "Decay Fit Parameter Map Display Range"=w21, "Decay Parameter Map X"=w19, "Decay Parameter Map Y"=w18, "Decay Parameter Map Value"=w17) -> (w24:T5)
  n11 = call "AlliGator Refnums Storage.vi"("Get(F)/Set"=TRUE, "AlliGator Refnum List"=AlliGator_Refnums_List."Decay Fit Parameter Map Ctrl Refnums", "Data in"=w24) -> ("Error Out"=w4:errorcluster)  [unwired: 7 in, 1 out]
  n12 = control-ref of="This VI"() -> (w2:refnum<vi>)
  n13 = call "AlliGator Store VI Refnum.vi"("error in (no error)"=w4, "VI Refnum"=w2) -> ("error out"=w3:errorcluster, "VI Refnum (dup)"=w1:refnum<vi>)  [unwired: 7 in, 1 out]
  n14 = call "Open VI Front Panel Hidden.vi"("error in"=w3, "VI in"=w1) -> ("error out"=w12:errorcluster, "VI out"=w9:refnum<vi>)  [unwired: 8 in]
  n15 = call "AlliGator Generic Image Display Mouse Move Flag.vi"("Image Control Refnum"=w5, "Flag (in)"=FALSE, "Read/Write"=Read-Write."Write") -> ()  [unwired: 6 in, 1 out]
  n16 = call "AlliGator subPanel User Event Refnum.vi"() -> ("subPanel Event"=w36:refnum<user-event>)  [unwired: 9 in]
  n17 = register-events(error in=w12, w36) -> (reference out=w35:refnum<event-registration>, error out=w11:errorcluster)  [unwired: 1 in]
  n18 = call "AlliGator Decay Fit Parameter Map Event Registration Refnums.vi"("error in (no error)"=w11) -> ("error out"=w10:errorcluster, "Decay Fit Parameter Map Display Event"=w13:refnum<event-registration>, "Decay Fit Parameter Map Display Range Event"=w14:refnum<event-registration>)  [unwired: 8 in]
  n19 = Bundle("Event Registration Refnum"=w35, "Decay Fit Parameter Map Display Range Event"=w14, "Decay Fit Parameter Map Display Event"=w13) -> (w31:T6)  [unwired: 1 in]
  n20 = call "Close Front Panel.vi"("error in (no error)"=w10, "VI in"=w9) -> ("VI out"=w8:refnum<vi>)  [unwired: 8 in, 1 out]
  n21 = call "AlliGator Queue.vi"() -> ("AlliGator Q"=w38:refnum<queue>)  [unwired: 8 in, 1 out]
  n22 = call "Get Notebook Queue.vi"() -> ("Notebook Queue"=w39:refnum<queue>)  [unwired: 9 in]
  n23 = while {
    tunnel: w39 -> [w50]
    tunnel: w38 -> [w47]
    tunnel: "AlliGator" ("Sender") -> [w45]
    tunnel: w8 -> [w43]
    tunnel: w31 -> [w42]
    tunnel: [w41] -> w34
    tunnel: [w40] -> w33
    stop <- w57 stop-if-true
    n24 = call "Busy Icon & Message Storage.vi"() -> ("Busy Icon Status (F = busy)"=w44:bool)  [unwired: 9 in, 2 out]
    n25 = event shown="[23] Panel Close?" {
      selector: w42 -> [_ _ _ _ _ _ _ _ _ _ _ _ _ _ w175 w188 _ w215 w238 _ w255 w272 _ _]
      dyn-events: [_ _ _ _ _ _ _ _ _ _ _ _ _ _ w174 w186 _ w214 w237 _ w256 w273 _ _] -> w41
      timeout: _ -> [_ _ _ _ _ _ _ _ _ _ _ _ _ _ _ _ _ _ _ _ _ _ _ _]
      tunnel: [_ w64 _ _ _ w78 w101 _ _ _ w154 w157 w159 _ w171 w184 _ _ _ _ _ _ _ w295] -> w51
      tunnel: [_ _ _ _ _ _ _ _ _ _ _ _ _ _ _ _ _ _ _ _ _ _ w287 _] -> w57
      tunnel: [_ _ _ _ _ _ w102 _ _ _ _ _ _ _ _ _ _ _ _ _ _ _ _ _] -> w48
      tunnel: [w59 _ _ _ _ _ w103 _ w140 w152 _ _ _ w163 _ _ w201 w217 _ w243 w260 w277 _ _] -> w46
      tunnel: w44 -> [w58 _ _ _ _ _ w104 _ w141 w151 _ _ _ w162 w172 w185 w199 w216 _ w242 w259 w276 _ _]
      tunnel: w45 -> [_ _ _ _ _ _ _ _ _ _ _ _ _ _ _ _ _ _ _ _ _ _ _ _]
      tunnel: w43 -> [_ _ _ _ _ _ _ _ _ _ w156 _ _ _ _ _ _ _ _ _ _ _ _ w294]
      event "Decay Fit Parameter Map Color Scale": Mouse Up {
        # "Replace with relevant action"
        n26 = event-data() -> ()  [unwired: 1 in, 1 out]
        n27 = case shown="True" w58 {
          tunnel: [_ w60] -> w59
          frame False {
          }
          frame True {
            n28 = Bundle By Name(cluster=T8 {"AlliGator Q Event"=enum."Phasor Plot:Change Phasor Plot Color Palette", "Data"=variant} ("element"), "Data"="Refresh Image" ("String")) -> (w62:T8)
            n29 = Build Array(w62) -> (w60:T8[])
          }
        }
      }
      event "Decay Fit Parameter Map Color Scale": Shortcut Menu Activation? {
        w67 = string[] ["Copy Color Scale to Clipboard", "-", "Change Display Format"] ("item names")
        n30 = event-data() -> ("MenuRef"=w65:refnum<k9>)  [unwired: 1 in]
        n31 = Delete Menu Items(9:w65) -> (0:w68:errorcluster, 3:w66:refnum<k9>)  [unwired: 3 in]
        n32 = Insert Menu Items(6:w68, 7:w67, 8:w67, 9:w66) -> (0:w64:errorcluster)  [unwired: 2 in, 2 out]
        n33 = event-data() -> ()  [unwired: 2 in, 1 out]
      }
      event "Decay Fit Parameter Map Color Scale": Shortcut Menu Selection (User) {
        n34 = event-data() -> ("CtlRef"=w70:refnum<vi>, "ItemTag"=w69:string)  [unwired: 1 in]
        n35 = case shown="\"Change Display Format\"" w69 {
          tunnel: w70 -> [_ w71 w72]
          frame "", Default {
          }
          frame "Copy Color Scale to Clipboard" {
            n36 = call "Export Color Ramp to Clipboard.vi"("ColorRamp Refnum"=w71) -> ()  [unwired: 11 in]
          }
          frame "Change Display Format" {
            n37 = call "Color Ramp Change Display Format.vi"("ColorRamp Refnum"=w72) -> ()  [unwired: 10 in, 1 out]
          }
        }
      }
      event "Decay Fit Parameter Map Display Range": Shortcut Menu Selection (User) {
        n38 = event-data() -> ("CtlRef"=w74:refnum<vi>, "ItemTag"=w73:string)  [unwired: 1 in]
        n39 = case shown="\"Change Display Format\"" w73 {
          tunnel: w74 -> [_ w75]
          frame "", Default {
          }
          frame "Change Display Format" {
            n40 = call "Slide Change Display Format.vi"("Slide Refnum"=w75) -> ()  [unwired: 10 in, 1 out]
          }
        }
      }
      event "Decay Fit Parameter Map Display": Mouse Wheel {
        n41 = event-data() -> ("CtlRef"=w77:refnum<vi>, "Delta"=w76:i32)  [unwired: 1 in]
        n42 = call "Image Display Mouse Wheel Zoom.vi"("Mouse Wheel Delta"=w76, "Image Control Refnum"=w77) -> ()  [unwired: 9 in, 1 out]
      }
      event "Decay Fit Parameter Map Display": Shortcut Menu Activation? {
        w93 = AlliGator_Variables_List."Decay Fit Parameter Map:Palette List" ("Alligator Variable")
        n43 = event-data() -> ("CtlRef"=w79:refnum<vi>, "MenuRef"=w80:refnum<k9>)  [unwired: 1 in]
        n44 = call "Alligator Variables Storage.vi"("Get(F)/Set"=FALSE, "AlliGator Variable"=AlliGator_Variables_List."Decay Fit Parameter Map:Palette Information" ("Alligator Variable")) -> ("Error Out"=w84:errorcluster, "Data out"=w83:variant)  [unwired: 7 in, 1 out]
        n45 = call "Alligator Variables Storage.vi"("Get(F)/Set"=FALSE, "AlliGator Variable"=w93) -> ("Error Out"=w96:errorcluster, "Data out"=w89:variant)  [unwired: 7 in, 1 out]
        n46 = Variant To Data(error in=w84, type=T10 {"Palette Name [# Colors,int?,inv?]"="", "Palette Type"=0, "Palette Colors"=[], "Interpolate?"=FALSE} ("Image Display Palette Information"), Variant=w83) -> (data=w85:T10, error out=w94:errorcluster)
        n47 = call-poly "Variant to Data.vi"("Variant"=w89) -> ("String Array"=w90:string[])  [unwired: 8 in]
        n48 = Unbundle By Name(w85) -> ("Palette Name [# Colors,int?,inv?]"=w87:string)
        n49 = Merge Errors(w94, w96) -> (w95:errorcluster)
        n50 = call "Check Selected Palette in Menu.vi"("Error In"=w95, "Palette List"=w90, "Checked Palette"=w87, "Menu in"=w80) -> ("Error Out"=w97:errorcluster, "Stored Palette List"=w92:string[], "menu reference out"=w98:refnum<k9>)  [unwired: 5 in]
        n51 = call "Alligator Variables Storage.vi"("Get(F)/Set"=TRUE, "AlliGator Variable"=w93, "Error In"=w97, "Data in"=w92) -> ("Error Out"=w99:errorcluster)  [unwired: 5 in, 2 out]
        n52 = call "AlliGator Add Python Functions to Object Menu.vi"("error in (no error)"=w99, "Menu in"=w98, "Object Refnum"=w79) -> ("error out"=w78:errorcluster)  [unwired: 6 in, 2 out]
        n53 = event-data() -> ()  [unwired: 2 in, 1 out]
      }
      event "Decay Fit Parameter Map Display": Shortcut Menu Selection (User) {
        n54 = event-data() -> ("CtlRef"=w108:refnum<vi>, "ItemTag"=w107:string, "ItemPath"=w106:string, "Coords"=w105:T16)  [unwired: 1 in]
        n55 = call "AlliGator Keyboard ID.vi"() -> ("keys pressed"=w100:T23)  [unwired: 9 in, 2 out]
        n56 = case shown="True" w104 {
          tunnel: w108 -> [_ w119]
          tunnel: w106 -> [_ w118]
          tunnel: w107 -> [_ w117]
          tunnel: [_ w116] -> w103
          tunnel: w105 -> [_ w115]
          tunnel: w100 -> [_ w111]
          tunnel: [_ w110] -> w102
          tunnel: [_ w109] -> w101
          frame False {
          }
          frame True {
            n57 = Index Array(array=w111) -> (element=w114:T13)  [unwired: 1 in]
            n58 = Equal?(x=w114, y=T13."H" ("element")) -> (x = y?=w112:bool)
            n59 = case shown="True" w112 {
              tunnel: w119 -> [w126 w132]
              tunnel: w118 -> [w124 _]
              tunnel: w117 -> [w125 w131]
              tunnel: [w128 _] -> w116
              tunnel: w115 -> [w123 _]
              tunnel: [_ w130] -> w110
              tunnel: [w121 w129] -> w109
              frame False {
                n60 = local read "Decay Fit Parameter"() -> (w120:T1)
                n61 = Bundle By Name(cluster=T14 {"Item Tag"="", "Image Control Refnum"=refnum, "Coords"={"Horizontal"=0, "Vertical"=0}, "Item Path"=""} ("Image Event Data"), "Image Control Refnum"=w126, "Item Tag"=w125, "Item Path"=w124, "Coords"=w123) -> (w122:T14)
                n62 = call "AlliGator Decay Fit Parameter Map Context Menu Handler.vi"("Decay Fit Parameter"=w120, "Image Event Data"=w122) -> ("Error Out"=w121:errorcluster, "AlliGator Actions"=w128:T8[])  [unwired: 8 in]
              }
              frame True {
                n63 = property class="ImageControl"(reference=w132) -> ("Label.Text"=w133:string)  [unwired: 1 in, 2 out]
                n64 = call "AlliGator Send Python Function Doc String to Notebook.vi"("Item Tag"=w131, "Target"=w133) -> ("Error Out"=w129:errorcluster, "Message"=w130:string)  [unwired: 8 in]
              }
            }
          }
        }
      }
      event "Decay Fit Parameter ROI Color": Value Change {
        n65 = event-data() -> ("NewVal"=w135:u32)  [unwired: 1 in]
        n66 = call <vilib>:"Color to RGB.vi"("Color"=w135) -> ("R"=w138:u8, "G"=w137:u8, "B"=w136:u8)  [unwired: 1 out]
        n67 = Bundle By Name(cluster=cluster{"Red":u8, "Green":u8, "Blue":u8} {"Red"=0, "Green"=0, "Blue"=0} ("ROI Color"), "Red"=w138, "Green"=w137, "Blue"=w136) -> (w134:cluster{"Red":u8, "Green":u8, "Blue":u8})
        n68 = property on="Decay Fit Parameter Map Display" class="ImageControl"("ROI Color"=w134) -> ()  [unwired: 2 in, 2 out]
      }
      event Value Change {
        n69 = event-data() -> ("NewVal"=w142:T1)  [unwired: 1 in]
        n70 = case shown="True" w141 {
          tunnel: w142 -> [_ w148]
          tunnel: [_ w143] -> w140
          frame False {
          }
          frame True {
            w145 = TRUE  # Parameter changed
            n71 = Bundle(cluster=T17 {"Parameter"=enum."Offset", "Parameter changed"=FALSE} ("output cluster"), "Parameter"=w148, "Parameter changed"=w145) -> (w146:T17)
            n72 = Bundle By Name(cluster=T8 {"AlliGator Q Event"=enum."Decay Fit Parameter Map:Build Decay Fit Parameter Map", "Data"=variant} ("Time-Gated Phasor Q Element"), "Data"=w146) -> (w149:T8)
            n73 = Build Array(w149, T8 {"AlliGator Q Event"=enum."Image:Update Image Profile Plots", "Data"=variant} ("Time-Gated Phasor Q Element")) -> (w143:T8[])
          }
        }
      }
      event "Overlay Decay Fit Parameter Map": Value Change {
        n74 = event-data() -> ()  [unwired: 1 in, 1 out]
        n75 = case shown="True" w151 {
          tunnel: [_ T8[] [{"AlliGator Q Event"=enum."Decay Fit Parameter Map:Overlay Decay Fit Parameter Map in Source Image", "Data"=variant}] ("element")] -> w152
          frame False {
          }
          frame True {
          }
        }
      }
      event "Pin Button": Value Change {
        n76 = event-data() -> ("NewVal"=w155:bool)  [unwired: 1 in]
        n77 = call "AlliGator Dock-Undock Subpanel Event.vi"("Dock?"=w155, "VI in"=w156) -> ("Error Out"=w154:errorcluster)  [unwired: 9 in]
      }
      event "Refresh Decay Fit Parameter Map": Shortcut Menu Activation? {
        n78 = event-data() -> ("MenuRef"=w158:refnum<k9>)  [unwired: 1 in]
        n79 = call "AlliGator Set Checks in Phasor Update Button.vi"("Menu in"=w158) -> ("Error Out"=w157:errorcluster)  [unwired: 10 in]
        n80 = event-data() -> ()  [unwired: 2 in, 1 out]
      }
      event "Refresh Decay Fit Parameter Map": Shortcut Menu Selection (User) {
        n81 = event-data() -> ("ItemTag"=w161:string, "CtlRef"=w160:refnum<vi>)  [unwired: 1 in]
        n82 = call "AlliGator Update Phasor Image Elements to Update.vi"("CtlRef"=w160, "Phasor Plot Element to Update"=w161) -> ("Error Out"=w159:errorcluster)  [unwired: 8 in, 1 out]
      }
      event "Refresh Decay Fit Parameter Map": Value Change {
        n83 = event-data() -> ()  [unwired: 1 in, 1 out]
        n84 = case shown="True" w162 {
          tunnel: [_ w164] -> w163
          frame False {
          }
          frame True {
            w167 = TRUE  # Parameter changed
            n85 = local read "Decay Fit Parameter"() -> (w166:T1)
            n86 = Bundle(cluster=T17 {"Parameter"=enum."Offset", "Parameter changed"=FALSE} ("output cluster"), "Parameter"=w166, "Parameter changed"=w167) -> (w165:T17)
            n87 = Bundle By Name(cluster=T8 {"AlliGator Q Event"=enum."Decay Fit Parameter Map:Build Decay Fit Parameter Map", "Data"=variant} ("Time-Gated Phasor Q Element"), "Data"=w165) -> (w169:T8)
            n88 = Build Array(w169) -> (w164:T8[])
          }
        }
      }
      event Mouse Enter {
        n89 = event-data() -> ("CtlRef"=w173:refnum<vi>)  [unwired: 1 in]
        n90 = case "Mouse Enter" shown="True" w172 {
          tunnel: [w176 w181] -> w174
          tunnel: w175 -> [w176 w180]
          tunnel: w173 -> [_ w177]
          tunnel: [_ w178] -> w171
          frame False {
          }
          frame True {
            n91 = Unbundle By Name(w180) -> ("Decay Fit Parameter Map Display Event"=w182:refnum<event-registration>)
            n92 = register-events(reference=w182, T15 refnum ("event source"), w177, w177, w177) -> (reference out=w183:refnum<event-registration>, error out=w178:errorcluster)  [unwired: 1 in]
            n93 = Bundle By Name(cluster=w180, "Decay Fit Parameter Map Display Event"=w183) -> (w181:T6)
          }
        }
      }
      event Mouse Leave {
        n94 = event-data() -> ("CtlRef"=w187:refnum<vi>)  [unwired: 1 in]
        n95 = case shown="True" w185 {
          tunnel: [w189 w194] -> w186
          tunnel: w188 -> [w189 w193]
          tunnel: w187 -> [_ w192]
          tunnel: [_ w191] -> w184
          frame False {
          }
          frame True {
            w190 = refnum<vi> refnum ("event source")
            n96 = Unbundle By Name(w193) -> ("Decay Fit Parameter Map Display Event"=w195:refnum<event-registration>)
            n97 = register-events(reference=w195, w192, w190, w190, w190) -> (reference out=w196:refnum<event-registration>, error out=w191:errorcluster)  [unwired: 1 in]
            n98 = Bundle By Name(cluster=w193, "Decay Fit Parameter Map Display Event"=w196) -> (w194:T6)
          }
        }
      }
      event Mouse Move {
        # "not busy and left button up"
        n99 = event-data() -> ("Time"=w203:u32, "CtlRef"=w202:refnum<vi>)  [unwired: 1 in]
        n100 = call "AlliGator Mouse ID.vi"() -> ("button info"=w200:T24)  [unwired: 8 in, 3 out]
        n101 = Unbundle By Name(w200) -> ("button 1"=w197:bool)
        n102 = Compound Arithmetic op=AND(w199, invert w197) -> (w198:bool)
        n103 = case shown="True" w198 {
          tunnel: w202 -> [_ w208]
          tunnel: [_ w204] -> w201
          tunnel: w203 -> [_ w210]
          frame False {
            # "if busy or the left button is down, do nothing"
          }
          frame True {
            w211 = T8 {"AlliGator Q Event"=enum."Decay Fit Parameter Map:Mouse Move", "Data"=variant} ("Array")
            n104 = call "AlliGator Filter Event.vi"("Time"=w210, "AlliGatorr Q Element"=w211) -> ("Filter Event?"=w207:bool)  [unwired: 8 in, 1 out]
            n105 = call "AlliGator Generic Image Display Mouse Move Flag.vi"("Image Control Refnum"=w208, "Read/Write"=Read-Write."Read") -> ("Flag (out)"=w206:bool)  [unwired: 7 in]
            n106 = Or(x=w207, y=w206) -> (x .or. y?=w205:bool)
            n107 = case shown="False" w205 {
              tunnel: w211 -> [w212 _]
              tunnel: w208 -> [_ _]
              tunnel: [w213 _] -> w204
              frame False {
                # "update X,Y,Value"
                n108 = Build Array(w212) -> (w213:T8[])
              }
              frame True {
                # "if not timed out AND action still unfolding, ignore event"
              }
            }
          }
        }
      }
      event Mouse Up {
        n109 = event-data() -> ("CtlRef"=w219:refnum<vi>, "PlatMods.Alt"=w218:bool)  [unwired: 1 in]
        n110 = case shown="True" w216 {
          tunnel: w219 -> [_ w225]
          tunnel: [_ w233] -> w217
          tunnel: w218 -> [_ w227]
          tunnel: w215 -> [w220 w223]
          tunnel: [w220 w221] -> w214
          frame False {
          }
          frame True {
            w224 = refnum<vi> refnum ("event source")
            n111 = Unbundle By Name(w223) -> ("Decay Fit Parameter Map Display Event"=w226:refnum<event-registration>)
            n112 = property class="ImageControl"(reference=w225) -> (reference out=w232:refnum<vi>, "ROI"=w231:T25, "Current ROI Tool"=w230:u32)  [unwired: 1 in, 1 out]
            n113 = Bundle By Name(cluster=T18 {"Current ROI Tool"=8, "ROI Descriptor"={"Global Rectangle"=[], "Contours"=[]}, "Shift"=FALSE, "Alt"=FALSE, "Image Display Refnum"=refnum} ("Phasor Plot Mouse Up Event Data"), "Image Display Refnum"=w232, "ROI Descriptor"=w231, "Current ROI Tool"=w230, "Alt"=w227) -> (w228:T18)
            n114 = register-events(reference=w226, w224, w224, w225, w225) -> (reference out=w222:refnum<event-registration>)  [unwired: 1 in, 1 out]
            n115 = Bundle By Name(cluster=w223, "Decay Fit Parameter Map Display Event"=w222) -> (w221:T6)
            n116 = Bundle By Name(cluster=T8 {"AlliGator Q Event"=enum."Decay Fit Parameter Map:Mouse Up", "Data"=variant} ("Array"), "Data"=w228) -> (w234:T8)
            n117 = Build Array(w234) -> (w233:T8[])
          }
        }
      }
      event Mouse Down {
        w241 = refnum<vi> refnum  # Slide (strict)
        n118 = event-data() -> ("CtlRef"=w236:refnum<vi>)  [unwired: 1 in]
        n119 = Unbundle By Name(w238) -> ("Decay Fit Parameter Map Display Range Event"=w240:refnum<event-registration>)
        n120 = register-events(reference=w240, w241, w236, w236, w236) -> (reference out=w239:refnum<event-registration>)  [unwired: 1 in, 1 out]
        n121 = Bundle By Name(cluster=w238, "Decay Fit Parameter Map Display Range Event"=w239) -> (w237:T6)
      }
      event Mouse Move {
        n122 = event-data() -> ("Time"=w244:u32)  [unwired: 1 in]
        n123 = case shown="True" w242 {
          tunnel: [_ w248] -> w243
          tunnel: w244 -> [_ w247]
          frame False {
          }
          frame True {
            w246 = T8 {"AlliGator Q Event"=enum."Decay Fit Parameter Map:Display Range Mouse Move", "Data"=variant} ("Time-Gated Phasor Q Element")
            n124 = call "AlliGator Filter Event.vi"("Time"=w247, "AlliGatorr Q Element"=w246) -> ("Filter Event?"=w245:bool)  [unwired: 8 in, 1 out]
            n125 = case shown="False" w245 {
              tunnel: [w251 _] -> w248
              tunnel: w246 -> [w250 _]
              frame False {
                n126 = local read "Decay Fit Parameter"() -> (w249:T1)
                n127 = Bundle By Name(cluster=w250, "Data"=w249) -> (w252:T8)
                n128 = Build Array(w252) -> (w251:T8[])
              }
              frame True {
              }
            }
          }
        }
      }
      event Mouse Leave {
        w253 = refnum<vi> refnum  # Slide (strict)
        n129 = event-data() -> ("Time"=w261:u32, "CtlRef"=w254:refnum<vi>)  [unwired: 1 in]
        n130 = Unbundle By Name(w255) -> ("Decay Fit Parameter Map Display Range Event"=w258:refnum<event-registration>)
        n131 = case shown="True" w259 {
          tunnel: [_ w265] -> w260
          tunnel: w261 -> [_ w264]
          frame False {
          }
          frame True {
            w263 = T8 {"AlliGator Q Event"=enum."Decay Fit Parameter Map:Display Range Mouse Move", "Data"=variant} ("Time-Gated Phasor Q Element")
            n132 = call "AlliGator Filter Event.vi"("Time"=w264, "AlliGatorr Q Element"=w263) -> ("Filter Event?"=w262:bool)  [unwired: 8 in, 1 out]
            n133 = case shown="False" w262 {
              tunnel: [w268 _] -> w265
              tunnel: w263 -> [w267 _]
              frame False {
                n134 = local read "Decay Fit Parameter"() -> (w266:T1)
                n135 = Bundle By Name(cluster=w267, "Data"=w266) -> (w269:T8)
                n136 = Build Array(w269) -> (w268:T8[])
              }
              frame True {
              }
            }
          }
        }
        n137 = register-events(reference=w258, w254, w253, w253, w253) -> (reference out=w257:refnum<event-registration>)  [unwired: 1 in, 1 out]
        n138 = Bundle By Name(cluster=w255, "Decay Fit Parameter Map Display Range Event"=w257) -> (w256:T6)
      }
      event Mouse Up {
        w270 = refnum<vi> refnum  # Slide (strict)
        n139 = event-data() -> ("Time"=w278:u32, "CtlRef"=w271:refnum<vi>)  [unwired: 1 in]
        n140 = Unbundle By Name(w272) -> ("Decay Fit Parameter Map Display Range Event"=w275:refnum<event-registration>)
        n141 = case shown="True" w276 {
          tunnel: [_ w282] -> w277
          tunnel: w278 -> [_ w281]
          frame False {
          }
          frame True {
            w280 = T8 {"AlliGator Q Event"=enum."Decay Fit Parameter Map:Display Range Mouse Move", "Data"=variant} ("Time-Gated Phasor Q Element")
            n142 = call "AlliGator Filter Event.vi"("Time"=w281, "AlliGatorr Q Element"=w280) -> ("Filter Event?"=w279:bool)  [unwired: 8 in, 1 out]
            n143 = case shown="False" w279 {
              tunnel: [w285 _] -> w282
              tunnel: w280 -> [w284 _]
              frame False {
                n144 = local read "Decay Fit Parameter"() -> (w283:T1)
                n145 = Bundle By Name(cluster=w284, "Data"=w283) -> (w286:T8)
                n146 = Build Array(w286) -> (w285:T8[])
              }
              frame True {
              }
            }
          }
        }
        n147 = register-events(reference=w275, w271, w270, w270, w270) -> (reference out=w274:refnum<event-registration>)  [unwired: 1 in, 1 out]
        n148 = Bundle By Name(cluster=w272, "Decay Fit Parameter Map Display Range Event"=w274) -> (w273:T6)
      }
      event User Event {
        n149 = event-data() -> ("subpanel"=w289:string, "event"=w288:string)  [unwired: 1 in]
        n150 = case shown="\"AlliGator\"" w289 {
          tunnel: w288 -> [_ w291]
          tunnel: [_ w290] -> w287
          frame "False", Default {
          }
          frame "AlliGator" {
            n151 = case shown="\"quit\"" w291 {
              tunnel: [_ TRUE] -> w290
              frame "False", Default {
              }
              frame "quit" {
              }
            }
          }
        }
      }
      event Panel Close? {
        w293 = TRUE ("Pin Button")
        n152 = event-data() -> ()  [unwired: 1 in, 1 out]
        n153 = property on="Pin Button" class="Bool (strict)"("Value"=w293) -> (error out=w296:errorcluster)  [unwired: 2 in, 1 out]
        n154 = call "AlliGator Dock-Undock Subpanel Event.vi"("Error In"=w296, "Dock?"=w293, "VI in"=w294) -> ("Error Out"=w295:errorcluster)  [unwired: 8 in]
        n155 = event-data("Discard?"=w293) -> ()  [unwired: 1 in, 1 out]
      }
    }
    n156 = call "AlliGator Settings Storage.vi"("AlliGator Settings List"=AlliGator_Settings_List."Miscellaneous:Verbose Error Mode") -> ("Variant Data out"=w56:variant)  [unwired: 9 in, 1 out]
    n157 = call-poly "Variant to Data.vi"("Variant"=w56) -> ("Value"=w49:bool)  [unwired: 8 in]
    n158 = call "Send Message to Notebook.vi"("Error In"=w51, "Text"=w48, "Notebook Queue"=w50) -> ("Error Out"=w53:errorcluster, "Notebook Queue"=w52:refnum<queue>)  [unwired: 5 in]
    n159 = call "Light Theme Message Style.vi"() -> ()  [unwired: 1 out]
    n160 = call "AlliGator Queue Non Empty Events.vi"("Actions"=w46, "AlliGator Q"=w47) -> ()  [unwired: 9 in, 1 out]
    n161 = call "Send Error to Notebook.vi"("error in (no error)"=w53, "Verbose Error Messages (T)"=w49, "State Machine Case Error Source"="Image Display Panel", "Notebook Q"=w52) -> ("Error Out"=w40:errorcluster)  [unwired: 7 in]
  }
  n162 = property on="Decay Fit Parameter ROI Color" class="ColBox"("Val(Sgnl)"="Decay Fit Parameter ROI Color") -> ()  [unwired: 2 in, 2 out]
  n163 = call "Tiny Clear Error.vi"("Error In"=w33) -> ("no Error Out"=w32:errorcluster)  [unwired: 8 in]
  n164 = Unregister For Events(event registration refnum=w34) -> (error out=w29:errorcluster)  [unwired: 1 in]
  n165 = invoke class="VI" method="FP.Close"(reference=w8, error in=w32) -> (error out=w30:errorcluster)  [unwired: 1 in, 2 out]
  n166 = Merge Errors(w30, w29) -> (w28:errorcluster)
  n167 = call "Tiny Clear Error.vi"("Error In"=w28) -> ()  [unwired: 8 in, 1 out]
